vi "Update Alias Name.vi"(7 "Alias Name Ref":refnum<vi>, 8 "error in (no error)":errorcluster, 11 "RESOURCE NAME Ref":refnum<vi>) -> (0 "error out":errorcluster, 3 "Alias Name":string)   [LabVIEW 2025, in "I2C Bus Monitor UI.lvlib"]
uses:
  I2C Bus Monitor UI.lvlib
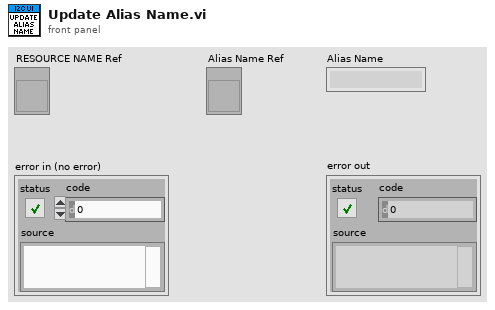
[diagram p1: front panel]
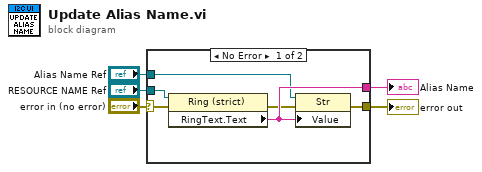
[diagram p0: block diagram]
diagram:
  n1 = case shown="No Error" "error in (no error)" {
    selector: "error in (no error)" -> [w8 w12]
    tunnel: [w11 _] -> w5
    tunnel: "Alias Name Ref" -> [w10 _]
    tunnel: "RESOURCE NAME Ref" -> [w7 _]
    tunnel: [w6 w12] -> w1
    frame No Error {
      n2 = property class="Ring (strict)"(reference=w7, error in=w8) -> (error out=w9:errorcluster, "RingText.Text"=w11:string)  [unwired: 1 out]
      n3 = property class="Str"(reference=w10, error in=w9, "Value"=w11) -> (error out=w6:errorcluster)  [unwired: 1 out]
    }
    frame Error {
    }
  }
  "error out" <- w1
  "Alias Name" <- w5
